vi "Update MCL.vi"(7 "initialize MCL value":bool, 8 "error in":errorcluster, 10 "MCL refnum":refnum<vi>, 11 "9210 in":refnum<class "9210.lvclass">) -> (0 "error out":errorcluster, 3 "9210 out":refnum<class "9210.lvclass">)   [LabVIEW 2020, in "Modules.lvlib" / "9210.lvclass"]
uses:
  9210.lvclass
  C:/Users/nitest/Desktop/Git 2020/niveristand-scan-engine-module-libraries/Source/RSI Module/RSI Module.lvclass
  9210.lvclass/9210.ctl
  <vilib>/Utility/miscctls.llb/LVRowAndColumnUnsignedTypeDef.ctl
  RSI Module/RSI Module.lvclass
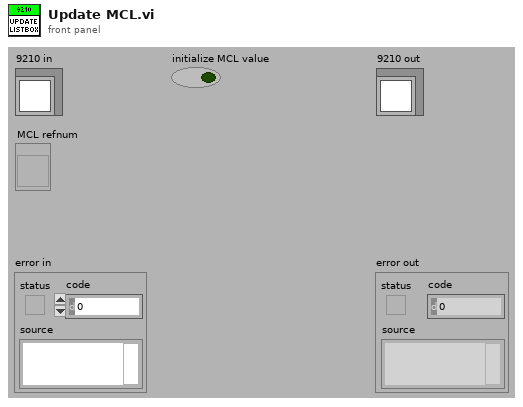
[diagram p1: front panel]
types:
  T1 = typedef "LVRowAndColumnUnsignedTypeDef.ctl" = cluster{"Row":u32, "Column":u32}
  T2 = typedef "Modules.lvlib/RSI Module.lvclass/Channels.ctl" = cluster{"# Input Channels":i32, "# Output Channels":i32, "Channel Type":T3, "Units":string}
  T3 = typedef "Modules.lvlib/RSI Module.lvclass/Channel Type.ctl" = enum16{"Analog", "Digital"}
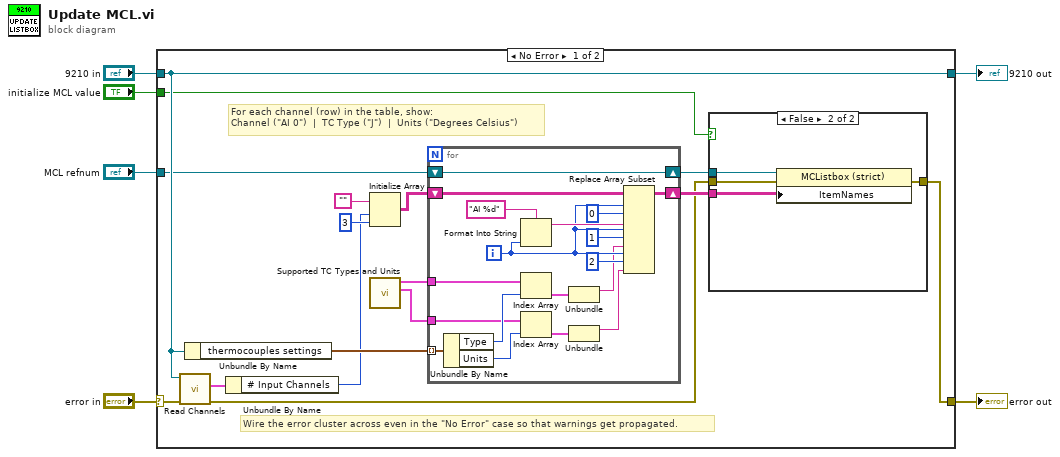
[diagram p0: block diagram]
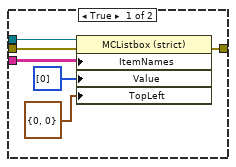
[diagram p2: hidden frame]
diagram:
  n1 = case shown="No Error" "error in" {
    selector: "error in" -> [w12 w52]
    tunnel: [w17 w52] -> w5
    tunnel: [w15 w51] -> w3
    tunnel: "9210 in" -> [w15 w51]
    tunnel: "MCL refnum" -> [w8 _]
    tunnel: "initialize MCL value" -> [w7 _]
    frame No Error {
      # "For each channel (row) in the table, show:\nChannel (\"AI 0\")  |  TC Type (\"J\")  |  Units (\"Degrees Celsius\")"
      # "Wire the error cluster across even in the \"No Error\" case so that warnings get propagated."
      n2 = call "Read Channels.vi"("error in (no error)"=w12, "RSI Module in"=w15) -> ("error out"=w11:errorcluster, "Channels"=w14:T2)  [unwired: 7 in, 1 out]
      n3 = Unbundle By Name(w15) -> ("thermocouples settings"=w16:cluster{"Units":u8, "Type":u8}[])
      n4 = Unbundle By Name(w14) -> ("# Input Channels"=w13:i32)
      n5 = Initialize Array("", w13, 3 ("dimension size")) -> (w20:string[][])
      n6 = call "Supported TC Types and Units.vi"() -> ("supported temperature units"=w10:cluster{"String":string, "Value":u16}[], "supported TC types"=w9:cluster{"String":string, "Value":u16}[])  [unwired: 10 in]
      n7 = for {
        shift-right: [w48] -> w22
        shift-left: w20 -> [w47]
        shift-right: [w50] -> w21
        shift-left: w8 -> [w50]
        tunnel: w16 -> [w35] mode=indexing
        tunnel: w9 -> [w34]
        tunnel: w10 -> [w33]
        i -> [w44]
        n8 = Unbundle By Name(w35) -> ("Type"=w37:u8, "Units"=w36:u8)
        n9 = Format Into String(format string="AI %d", w44) -> (resulting string=w45:string)  [unwired: 2 in, 1 out]
        n10 = Index Array(array=w34, index=w37) -> (element=w42:cluster{"String":string, "Value":u16})
        n11 = Index Array(array=w33, index=w36) -> (element=w41:cluster{"String":string, "Value":u16})
        n12 = Unbundle(w42) -> ("String"=w39:string)  [unwired: 1 out]
        n13 = Unbundle(w41) -> ("String"=w38:string)  [unwired: 1 out]
        n14 = Replace Array Subset(array=w47, new element #1=w45, index (row) #1=w44, index (col) #1=0 ("Column 1"), new element #2=w39, index (row) #2=w44, index (col) #2=1 ("Column 1"), new element #3=w38, index (row) #3=w44, index (col) #3=2 ("disabled index (col)")) -> (w48:string[][])
      }
      n15 = case shown="False" w7 {
        tunnel: w22 -> [w28 w32]
        tunnel: w21 -> [w27 w31]
        tunnel: [w26 w30] -> w17
        tunnel: w11 -> [w23 w29]
        frame True {
          n16 = property on="Property Node" class="MCListbox (strict)"(reference=w27, error in=w23, "ItemNames"=w28, "Value"=i32[] [0], "TopLeft"=T1 {"Row"=0, "Column"=0} ("Top Left Visible Cell")) -> (error out=w26:errorcluster)  [unwired: 1 out]
        }
        frame False {
          n17 = property on="Property Node" class="MCListbox (strict)"(reference=w31, error in=w29, "ItemNames"=w32) -> (error out=w30:errorcluster)  [unwired: 1 out]
        }
      }
    }
    frame Error {
    }
  }
  "error out" <- w5
  "9210 out" <- w3
